vi "lvmcp_geterrors.vi"() -> ()   [LabVIEW 2026]
panel:
  out "Details":string[](array[string])
  out "Errors":string[](array[string])
  out "error out":errorcluster
  in  "reference":refnum<vi>
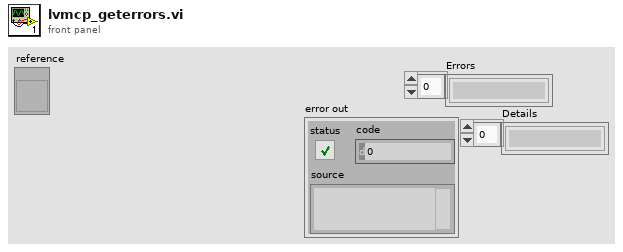
[diagram p1: front panel]
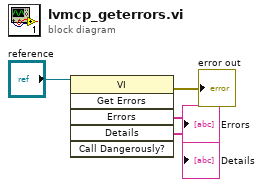
[diagram p0: block diagram]
diagram:
  n1 = invoke class="VI" method="Get Errors"(reference="reference") -> (error out=→"error out":errorcluster, "Errors"=→"Errors":string[], "Details"=→"Details":string[])  [unwired: 5 in, 3 out]
